vi "Callback Change Node Path.vi"(6 "Variant":variant, 8 "error in (no error)":errorcluster, 9 "Old values":string[][](array[string]), 10 "object ref in":T1, 11 "Table Change":T2) -> (0 "error out":errorcluster)   [LabVIEW 2014, in "OPC UA Client editor node.lvclass"]
uses:
  OPC UA Client editor node.lvclass
  <vilib>/NI/DCAF/Tag Editor Core/Table API/Table Manager/Cell Change.ctl
  <vilib>/NI/DCAF/Tag Editor Core/Table API/Table Manager/object ref.ctl
  <vilib>/NI/DCAF/Tag Editor Core/Configuration Editor/Classes/Engine Parent/Engine Parent Editor Node.lvclass
  <vilib>/NI/DCAF/Tag Editor Core/Configuration Editor/Classes/Module editor node/module editor node.lvclass
  module/configuration/OPC UA Client configuration.lvclass
  module/configuration/OPC UA Client configuration.lvclass/OPC UA Client configuration.ctl
  <vilib>/NI/Tag Bus Module Framework/channel/TBM channel.lvclass
  <vilib>/NI/DCAF/Tag Editor Core/Table API/Table Manager.lvlib
  <vilib>/NI/DCAF/Tag Editor Core/Table API/Table Manager/Table Manager.lvclass
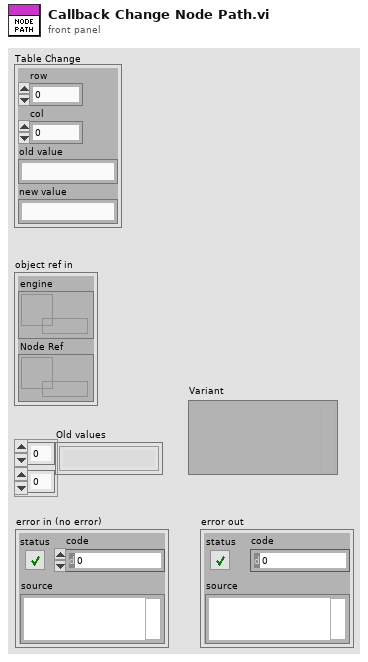
[diagram p1: front panel]
types:
  T1 = typedef "Table Manager.lvlib/Table Manager.lvclass/object ref.ctl" = cluster{"engine":refnum<data-value>, "Node Ref":refnum<data-value>}
  T2 = typedef "Table Manager.lvlib/Cell Change.ctl" = cluster{"row":i32, "col":i32, "old value":string, "new value":string}
  T3 = typedef "OPC UA Client configuration.lvclass/Line.ctl" = cluster{"channel":refnum<class "TBM channel.lvclass">, "Node Path":string, "OPC UA Data Type":T4}
  T4 = typedef "OPC UA Client configuration.lvclass/OPC UA Data Type.ctl" = u16
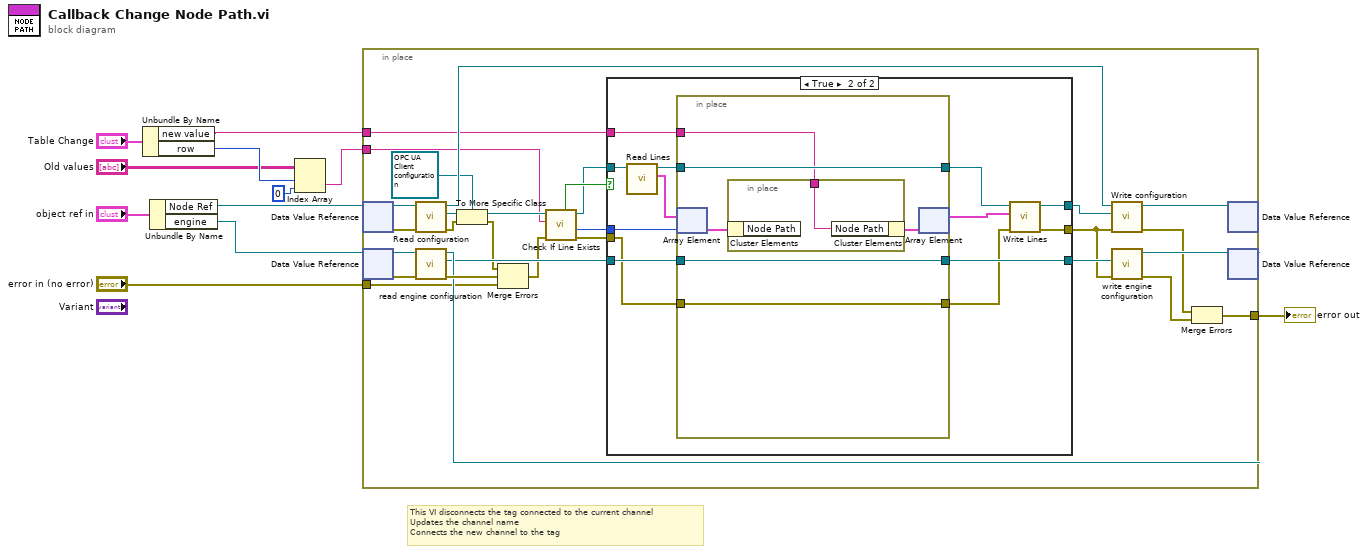
[diagram p0: block diagram]
diagram:
  # "This VI disconnects the tag connected to the current channel\nUpdates the channel name\nConnects the new channel to the tag"
  n1 = Unbundle By Name("Table Change") -> ("new value"=w5:string, "row"=w4:i32)
  n2 = Unbundle By Name("object ref in") -> ("Node Ref"=w8:refnum<data-value>, "engine"=w7:refnum<data-value>)
  n3 = Index Array(array="Old values", index (row)=w4, index (col)=0 ("disabled index (col)")) -> (element=w1:string)
  n4 = in-place {
    in-place-border: [w32] -> w11
    in-place-border: "error in (no error)" -> [w28]
    in-place-border: w1 -> [w12]
    in-place-border: w5 -> [w24]
    n5 = in-place-dvr #1(w8) -> (w22:refnum<class "module editor node.lvclass">, w31:errorcluster)
    n6 = in-place-dvr #2(w7) -> (w39:refnum<class "Engine Parent Editor Node.lvclass">, w40:errorcluster)
    n7 = call-dynamic "Read configuration.vi"("error in"=w31, "NISE_CEF_serializable node in"=w22) -> ("error out"=w14:errorcluster, "configuration"=w29:refnum<class "NISE_CEF_serializable configuration.lvclass">, "NISE_CEF_serializable node out"=w30:refnum<class "module editor node.lvclass">)  [unwired: 7 in]
    n8 = call <vilib>:"read engine configuration.vi"("error in"=w40, "Engine Parent Editor Node in"=w39) -> ("error out"=w36:errorcluster, "engine configuration"=w19:refnum<class "engine configuration.lvclass">, "Engine Parent Editor Node out"=w35:refnum<class "Engine Parent Editor Node.lvclass">)  [unwired: 7 in]
    n9 = To More Specific Class(target class=refnum<class "OPC UA Client configuration.lvclass"> refnum ("tag bus configurable plugin module configuration"), reference=w29, error in=w14) -> (specific class reference=w21:refnum<class "OPC UA Client configuration.lvclass">, error out=w13:errorcluster)
    n10 = Merge Errors(w13, w36, w28) -> (w17:errorcluster)
    n11 = call-dynamic "Check If Line Exists.vi"("error in"=w17, "name to locate"=w12, "OPC UA configuration in"=w21) -> ("error out"=w18:errorcluster, "index"=w25:i32, "OPC UA configuration out"=w16:refnum<class "OPC UA Client configuration.lvclass">, "found?"=w23:bool)  [unwired: 4 in, 1 out]
    n12 = case shown="True" w23 {
      tunnel: [w43 w56] -> w26
      tunnel: w16 -> [w43 w55]
      tunnel: w25 -> [_ w52]
      tunnel: w24 -> [_ w51]
      tunnel: w19 -> [w42 w50]
      tunnel: [w42 w49] -> w20
      tunnel: [w41 w48] -> w15
      tunnel: w18 -> [w41 w46]
      frame False {
      }
      frame True {
        n13 = call "Read Lines.vi"("OPC UA configuration in"=w55) -> ("Lines"=w54:T3[], "OPC UA configuration out"=w45:refnum<class "OPC UA Client configuration.lvclass">)  [unwired: 8 in, 1 out]
        n14 = in-place {
          in-place-border: w51 -> [w59]
          in-place-border: w50 -> [w62]
          in-place-border: [w62] -> w49
          in-place-border: [w57] -> w47
          in-place-border: w46 -> [w57]
          in-place-border: w45 -> [w61]
          in-place-border: [w61] -> w44
          n15 = in-place-array #3(w54, w52) -> (w60:T3)
          n16 = in-place {
            in-place-border: w59 -> [w63]
            n17 = in-place-cluster #4(w60) -> ()  [unwired: 1 out]
            n18 = in-place-cluster #4("Node Path"=w63) -> (w58:T3)
          }
          n19 = in-place-array #3(w58) -> (w53:T3[])  [unwired: 1 out]
        }
        n20 = call "Write Lines.vi"("error in (no error)"=w47, "Lines"=w53, "OPC UA configuration in"=w44) -> ("error out"=w48:errorcluster, "OPC UA configuration out"=w56:refnum<class "OPC UA Client configuration.lvclass">)  [unwired: 7 in]
      }
    }
    n21 = call-dynamic "Write configuration.vi"("error in"=w15, "configuration"=w26, "NISE_CEF_serializable node in"=w30) -> ("error out"=w33:errorcluster, "NISE_CEF_serializable node out"=w37:refnum<class "module editor node.lvclass">)  [unwired: 7 in]
    n22 = call <vilib>:"write engine configuration.vi"("error in"=w15, "engine configuration"=w20, "Engine Parent Editor Node in"=w35) -> ("error out"=w34:errorcluster, "Engine Parent Editor Node out"=w38:refnum<class "Engine Parent Editor Node.lvclass">)  [unwired: 7 in]
    n23 = Merge Errors(w33, w34) -> (w32:errorcluster)
    n24 = in-place-dvr #1(w37) -> ()  [unwired: 2 out]
    n25 = in-place-dvr #2(w38) -> ()  [unwired: 2 out]
  }
  "error out" <- w11
